vi "Close References.vi"(8 "error in":errorcluster, 11 "Project Manager in":refnum<class "Project Manager.lvclass">) -> (0 "error out":errorcluster, 3 "Project Manager out":refnum<class "Project Manager.lvclass">)   [LabVIEW 2026, in "Project Manager.lvclass"]
doc: "Close all project references."
uses:
  Project Manager.lvclass
  Project Manager.lvclass/Project Manager.ctl
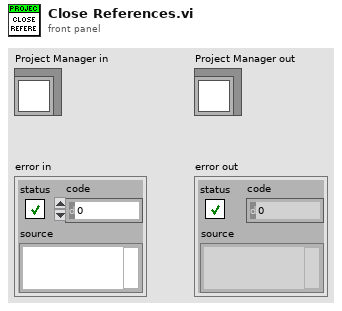
[diagram p1: front panel]
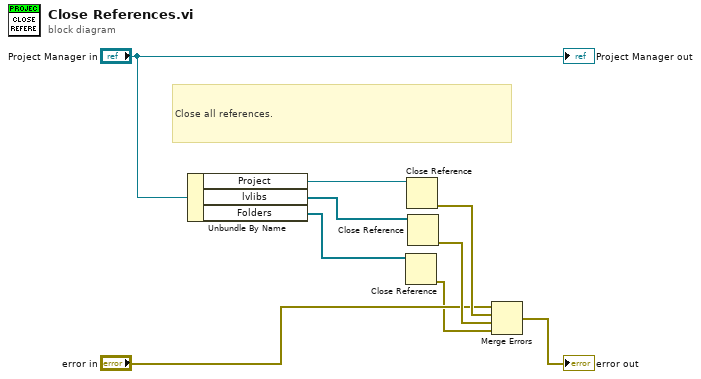
[diagram p0: block diagram]
diagram:
  # "Close all references."
  n1 = Unbundle By Name("Project Manager in") -> ("Project"=w3:refnum<vi>, "lvlibs"=w2:refnum<vi>[], "Folders"=w1:refnum<vi>[])
  n2 = Close Reference(reference=w1) -> (error out=w5:errorcluster)  [unwired: 1 in]
  n3 = Close Reference(reference=w3) -> (error out=w8:errorcluster)  [unwired: 1 in]
  n4 = Close Reference(reference=w2) -> (error out=w9:errorcluster)  [unwired: 1 in]
  n5 = Merge Errors("error in", w8, w9, w5) -> (→"error out":errorcluster)
  "Project Manager out" <- "Project Manager in"
